vi "Serializer Factory.vi"(8 "error in (no error)":errorcluster, 11 "Display Format":T1) -> (0 "error out":errorcluster, 3 "Serializer":refnum<class "Serializer.lvclass">)   [LabVIEW 2017, in "Serializer.lvlib" / "Serializer.lvclass"]
doc: "Factory to load the proper Serializer based on the <b>Display Format</b>."
uses:
  Serializer/Serializer.lvclass
  Serializer/Type Defs/Display Format.ctl
  Serializer/Serializer.lvlib
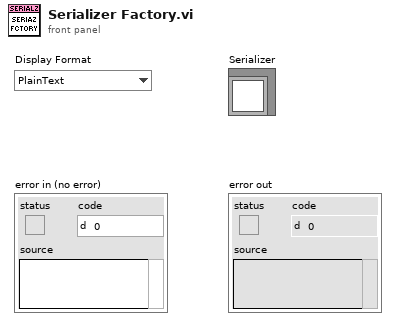
[diagram p1: front panel]
types:
  T1 = typedef "Serializer.lvlib/Display Format.ctl" = enum16{"PlainText", "PlainText.INI", "XML", "JSON"}
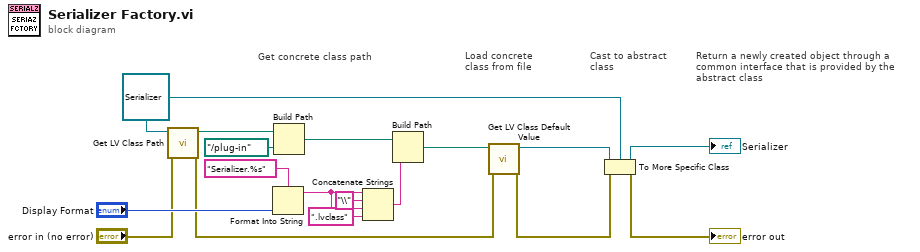
[diagram p0: block diagram]
diagram:
  w3 = refnum<class "Serializer.lvclass"> refnum ("Error Log.lvlib:Serializer.lvclass")
  # "Return a newly created object through a common interface that is provided by the abstract class"
  # "Get concrete class path"
  # "Cast to abstract class"
  # "Load concrete class from file"
  n1 = call <vilib>:"Get LV Class Path.vi"("error in (no error)"="error in (no error)", "object"=w3) -> ("error out"=w1:errorcluster, "class path"=w13:path)  [unwired: 8 in]
  n2 = Format Into String(format string="Serializer.%s", "Display Format") -> (resulting string=w7:string)  [unwired: 2 in, 1 out]
  n3 = Build Path(base path=w13, name or relative path=path "../plug-in") -> (appended path=w9:path)
  n4 = Concatenate Strings(w7, "\\" ("string"), w7, ".lvclass" ("string")) -> (w8:string)
  n5 = Build Path(base path=w9, name or relative path=w8) -> (appended path=w4:path)
  n6 = call <vilib>:"Get LV Class Default Value.vi"("error in (no error)"=w1, "class path"=w4) -> ("error out"=w16:errorcluster, "object"=w17:refnum<class>)  [unwired: 8 in]
  n7 = To More Specific Class(target class=w3, reference=w17, error in=w16) -> (specific class reference=→"Serializer":refnum<class "Serializer.lvclass">, error out=→"error out":errorcluster)
